vi "Creation_segment EPC3000.vi"(1 "Valeur 2":dbl format="%#.1f", 2 "Valeur 1":dbl format="%#.1f", 3 "Type de segment/Valeur 0":u8, 4 "Numéro de segment":u8) -> (0 "Segment":cluster{"chaîne p":string, "Valeur 1":dbl}[](array[cluster]) {"Valeur 1" format="%#.1f"})   [LabVIEW 2022 SP3]
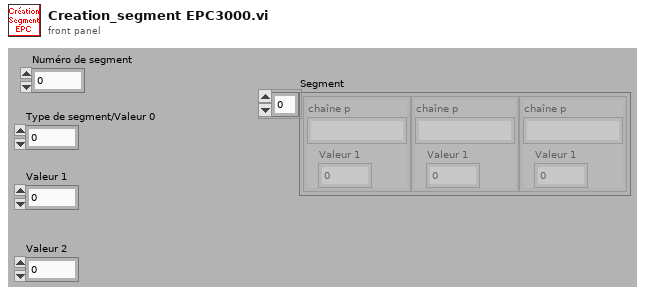
[diagram p1: front panel]
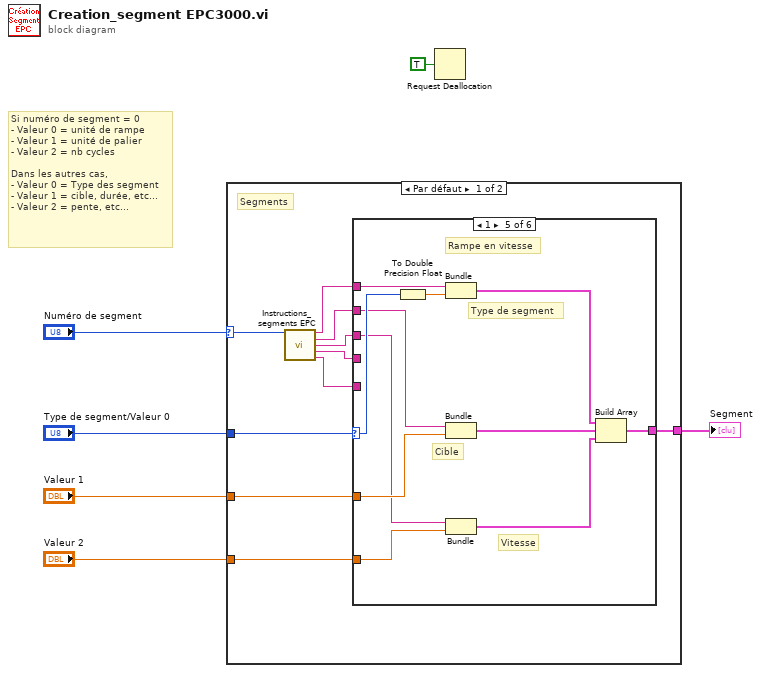
[diagram p0: block diagram]
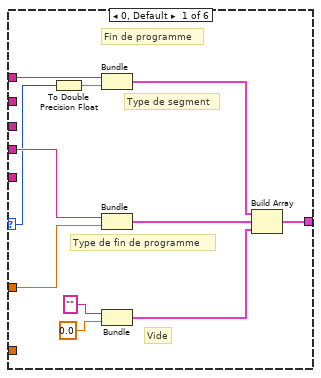
[diagram p2: hidden frame]
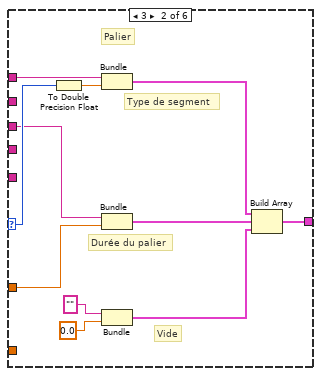
[diagram p3: hidden frame]
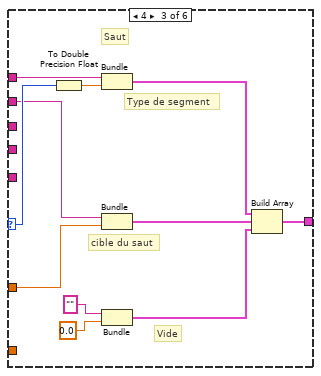
[diagram p4: hidden frame]
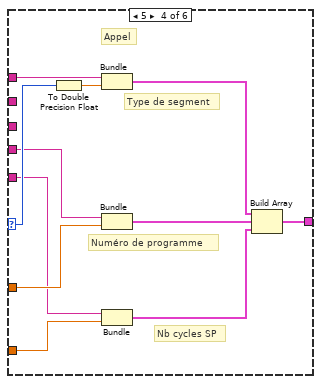
[diagram p5: hidden frame]
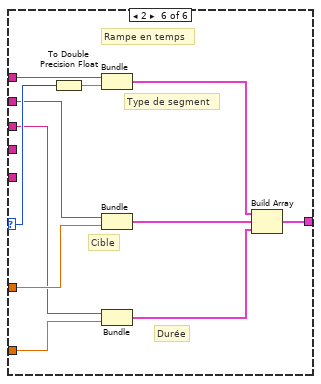
[diagram p6: hidden frame]
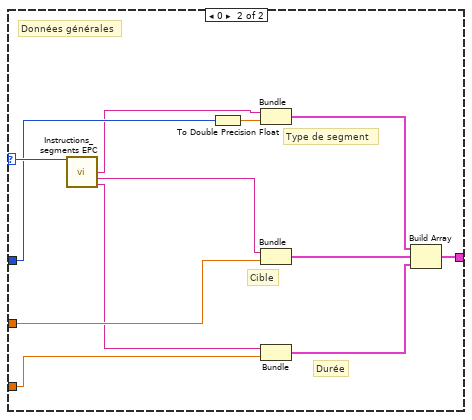
[diagram p7: hidden frame]
diagram:
  # "Si numéro de segment = 0\n- Valeur 0 = unité de rampe\n- Valeur 1 = unité de palier\n- Valeur 2 = nb cycles\n\nDans les autres cas,\n- Valeur 0 = Type des segment\n- Valeur 1 = cible, durée, etc...\n- Valeur 2 = pente, etc..."
  n1 = case shown="Par défaut" "Numéro de segment" {
    selector: "Numéro de segment" -> [w7 w94]
    tunnel: "Type de segment/Valeur 0" -> [w16 w88]
    tunnel: "Valeur 1" -> [w15 w87]
    tunnel: "Valeur 2" -> [w14 w86]
    tunnel: [w8 w89] -> w3
    frame Default {
      # "Segments"
      n2 = call "Instructions_segments EPC.vi"("Numéro de segment"=w7) -> ("chaîne $"=w13:string, "chaîne s"=w12:string, "chaîne d"=w11:string, "chaîne p"=w10:string, "chaîne o"=w9:string)  [unwired: 10 in]
      n3 = case shown="1" w16 {
        selector: w16 -> [w17 w29 w40 w53 w64 w75]
        tunnel: w15 -> [w23 w35 w46 w57 w68 w79]
        tunnel: w14 -> [_ _ _ w51 w63 w74]
        tunnel: w13 -> [w27 w38 w49 w60 w71 w82]
        tunnel: w12 -> [_ _ w39 _ w62 w73]
        tunnel: w11 -> [_ w28 _ _ w61 w72]
        tunnel: w10 -> [w26 _ _ w52 _ _]
        tunnel: w9 -> [_ _ _ w50 _ _]
        tunnel: [w22 w34 w45 w56 w67 w78] -> w8
        frame 0, Default {
          # "Vide"
          # "Type de fin de programme"
          # "Type de segment"
          # "Fin de programme"
          n4 = To Double Precision Float(number=w17) -> (double precision float=w18:dbl)
          n5 = Bundle("chaîne $"=w27, w18) -> (w25:cluster{"chaîne $":string, dbl})  [unwired: 1 in]
          n6 = Bundle("chaîne p"=w26, "Valeur 1"=w23) -> (w24:cluster{"chaîne p":string, "Valeur 1":dbl})  [unwired: 1 in]
          n7 = Bundle("chaîne p"="", "Valeur 1"=0.0) -> (w21:cluster{"chaîne p":string, "Valeur 1":dbl})  [unwired: 1 in]
          n8 = Build Array(w25, w24, w21) -> (w22:cluster{"chaîne p":string, "Valeur 1":dbl}[])
        }
        frame 3 {
          # "Vide"
          # "Durée du palier"
          # "Type de segment"
          # "Palier"
          n9 = To Double Precision Float(number=w29) -> (double precision float=w30:dbl)
          n10 = Bundle("chaîne $"=w38, w30) -> (w37:cluster{"chaîne $":string, dbl})  [unwired: 1 in]
          n11 = Bundle("chaîne d"=w28, "Valeur 1"=w35) -> (w36:cluster{"chaîne d":string, "Valeur 1":dbl})  [unwired: 1 in]
          n12 = Bundle("chaîne p"="", "Valeur 1"=0.0) -> (w33:cluster{"chaîne p":string, "Valeur 1":dbl})  [unwired: 1 in]
          n13 = Build Array(w37, w36, w33) -> (w34:cluster{"chaîne p":string, "Valeur 1":dbl}[])
        }
        frame 4 {
          # "Vide"
          # "cible du saut"
          # "Type de segment"
          # "Saut"
          n14 = To Double Precision Float(number=w40) -> (double precision float=w41:dbl)
          n15 = Bundle("chaîne $"=w49, w41) -> (w48:cluster{"chaîne $":string, dbl})  [unwired: 1 in]
          n16 = Bundle("chaîne s"=w39, "Valeur 1"=w46) -> (w47:cluster{"chaîne s":string, "Valeur 1":dbl})  [unwired: 1 in]
          n17 = Bundle("chaîne p"="", "Valeur 1"=0.0) -> (w44:cluster{"chaîne p":string, "Valeur 1":dbl})  [unwired: 1 in]
          n18 = Build Array(w48, w47, w44) -> (w45:cluster{"chaîne p":string, "Valeur 1":dbl}[])
        }
        frame 5 {
          # "Nb cycles SP"
          # "Numéro de programme"
          # "Type de segment"
          # "Appel"
          n19 = To Double Precision Float(number=w53) -> (double precision float=w54:dbl)
          n20 = Bundle("chaîne $"=w60, w54) -> (w59:cluster{"chaîne $":string, dbl})  [unwired: 1 in]
          n21 = Bundle("chaîne p"=w52, "Valeur 1"=w57) -> (w58:cluster{"chaîne p":string, "Valeur 1":dbl})  [unwired: 1 in]
          n22 = Bundle("chaîne o"=w50, "Valeur 2"=w51) -> (w55:cluster{"chaîne o":string, "Valeur 2":dbl})  [unwired: 1 in]
          n23 = Build Array(w59, w58, w55) -> (w56:cluster{"chaîne o":string, "Valeur 2":dbl}[])
        }
        frame 1 {
          # "Vitesse"
          # "Cible"
          # "Type de segment"
          # "Rampe en vitesse"
          n24 = To Double Precision Float(number=w64) -> (double precision float=w65:dbl)
          n25 = Bundle("chaîne $"=w71, w65) -> (w70:cluster{"chaîne $":string, dbl})  [unwired: 1 in]
          n26 = Bundle("chaîne s"=w62, "Valeur 1"=w68) -> (w69:cluster{"chaîne s":string, "Valeur 1":dbl})  [unwired: 1 in]
          n27 = Bundle("chaîne d"=w61, "Valeur 2"=w63) -> (w66:cluster{"chaîne d":string, "Valeur 2":dbl})  [unwired: 1 in]
          n28 = Build Array(w70, w69, w66) -> (w67:cluster{"chaîne d":string, "Valeur 2":dbl}[])
        }
        frame 2 {
          # "Durée"
          # "Cible"
          # "Type de segment"
          # "Rampe en temps"
          n29 = To Double Precision Float(number=w75) -> (double precision float=w76:dbl)
          n30 = Bundle("chaîne $"=w82, w76) -> (w81:cluster{"chaîne $":string, dbl})  [unwired: 1 in]
          n31 = Bundle("chaîne s"=w73, "Valeur 1"=w79) -> (w80:cluster{"chaîne s":string, "Valeur 1":dbl})  [unwired: 1 in]
          n32 = Bundle("chaîne d"=w72, "Valeur 2"=w74) -> (w77:cluster{"chaîne d":string, "Valeur 2":dbl})  [unwired: 1 in]
          n33 = Build Array(w81, w80, w77) -> (w78:cluster{"chaîne d":string, "Valeur 2":dbl}[])
        }
      }
    }
    frame 0 {
      # "Durée"
      # "Cible"
      # "Type de segment"
      # "Données générales"
      n34 = call "Instructions_segments EPC.vi"("Numéro de segment"=w94) -> ("chaîne d"=w83:string, "chaîne p"=w84:string, "chaîne o"=w85:string)  [unwired: 10 in, 2 out]
      n35 = To Double Precision Float(number=w88) -> (double precision float=w90:dbl)
      n36 = Bundle("chaîne d"=w83, w90) -> (w93:cluster{"chaîne d":string, dbl})  [unwired: 1 in]
      n37 = Bundle("chaîne p"=w84, "Valeur 1"=w87) -> (w92:cluster{"chaîne p":string, "Valeur 1":dbl})  [unwired: 1 in]
      n38 = Bundle("chaîne o"=w85, "Valeur 2"=w86) -> (w91:cluster{"chaîne o":string, "Valeur 2":dbl})  [unwired: 1 in]
      n39 = Build Array(w93, w92, w91) -> (w89:cluster{"chaîne o":string, "Valeur 2":dbl}[])
    }
  }
  "Segment" <- w3
  n40 = Request Deallocation(TRUE ("flag")) -> ()
